vi "Controlword_ModeSpecific_VelocityProfile.vi"(7 "Halt":bool, 10 "New Setpoint?":bool, 11 "ControlWord In":u16 format="%08b") -> (3 "ControlWord Out":u16 format="%08b")   [LabVIEW 2017, in "WordManipulationLibrary.lvlib"]
uses:
  WordManipulationLibrary.lvlib
  Bit Manipulation.lvlib
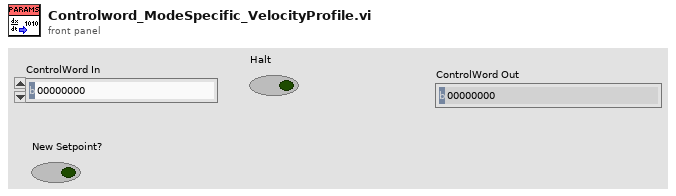
[diagram p1: front panel]
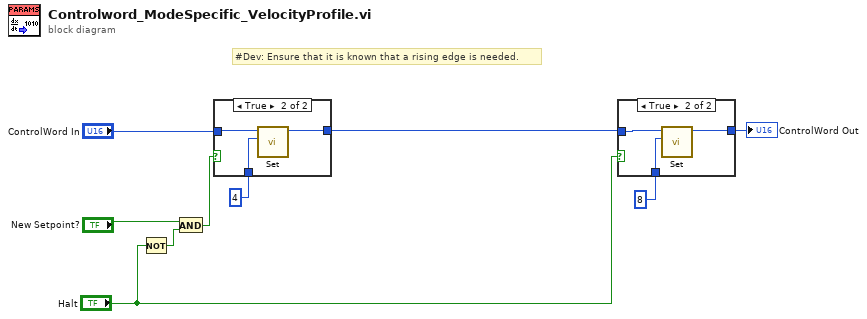
[diagram p0: block diagram]
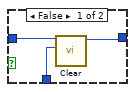
[diagram p2: hidden frame]
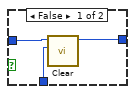
[diagram p3: hidden frame]
diagram:
  # "#Dev: Ensure that it is known that a rising edge is needed."
  n1 = Not(x="Halt") -> (.not. x?=w3:bool)
  n2 = And(x="New Setpoint?", y=w3) -> (x .and. y?=w2:bool)
  n3 = case shown="True" w2 {
    tunnel: "ControlWord In" -> [w12 w15]
    tunnel: [w11 w14] -> w1
    tunnel: u8 4 ("Bit to set") -> [w10 w13]
    frame False {
      n4 = call "Clear.vi"("Bit to clear"=w10, "Data_In"=w12) -> ("Data_Out"=w11:u16)  [unwired: 9 in]
    }
    frame True {
      n5 = call "Set.vi"("Bit to set"=w13, "Data_In"=w15) -> ("Data_Out"=w14:u16)  [unwired: 9 in]
    }
  }
  n6 = case shown="True" "Halt" {
    tunnel: w1 -> [w17 w20]
    tunnel: [w16 w21] -> w8
    tunnel: u8 8 ("Bit to set") -> [w18 w19]
    frame False {
      n7 = call "Clear.vi"("Bit to clear"=w18, "Data_In"=w17) -> ("Data_Out"=w16:u16)  [unwired: 9 in]
    }
    frame True {
      n8 = call "Set.vi"("Bit to set"=w19, "Data_In"=w20) -> ("Data_Out"=w21:u16)  [unwired: 9 in]
    }
  }
  "ControlWord Out" <- w8
